vi "UE_Relative_Target.vi"(1 "offset_mm":dbl, 2 "reference_mm":dbl) -> (0 "target_mm":dbl)   [LabVIEW 2026]
doc: "INTENT: Calculate PC lever target from measured servo position and configurable relative displacement. INPUTS: reference_mm (double), offset_mm (double). OUTPUTS: target_mm (double). DESIGN CONSTRAINT: Reference is servo encoder-based calibrated lever position, not hydraulic hitch feedback. REQUIREMENTS: SRS-F-020. No physical hardware side effects. Acceptance requires native LabVIEW compilation and behavioral testing."
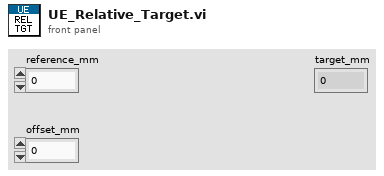
[diagram p1: front panel]
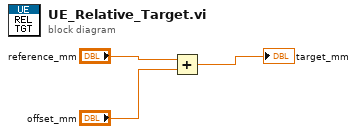
[diagram p0: block diagram]
diagram:
  n1 = Add(x="reference_mm", y="offset_mm") -> (x+y=→"target_mm":dbl)
